vi "Unflatten Buffer Configuration.vi"(11 "Flattened Configuration":u8[](array[numeric]) format="%.0x") -> (3 "Buffer Configuration":T1)   [LabVIEW 2021, in "CIF_Iceoryx_PCAP_Universal.lvclass"]
uses:
  CIF_Iceoryx_PCAP_Universal.lvclass
  Typedef/Buffer Configuration Data.ctl
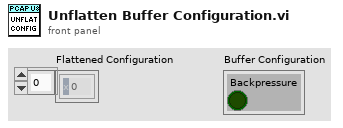
[diagram p1: front panel]
types:
  T1 = typedef "CIF_Iceoryx_PCAP_Universal.lvclass/Buffer Configuration Data.ctl" = cluster{"Backpressure":bool}
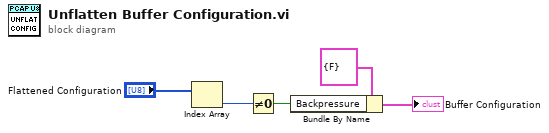
[diagram p0: block diagram]
diagram:
  n1 = Index Array(array="Flattened Configuration") -> (element=w2:u8)  [unwired: 1 in]
  n2 = Not Equal To 0?(x=w2) -> (x != 0?=w1:bool)
  n3 = Bundle By Name(cluster=T1 {"Backpressure"=FALSE} ("Buffer Configuration"), "Backpressure"=w1) -> (→"Buffer Configuration":T1)
